vi "xnet_canopen_create.vi"(8 "error in (no error)":errorcluster) -> (0 "error out":errorcluster, 3 "xnet_co_handle":u64)   [LabVIEW 2023, in "xnet_canopen.lvlib"]
uses:
  xnet_canopen.lvlib
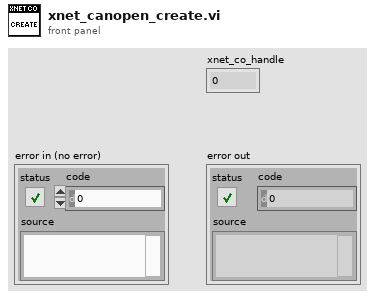
[diagram p1: front panel]
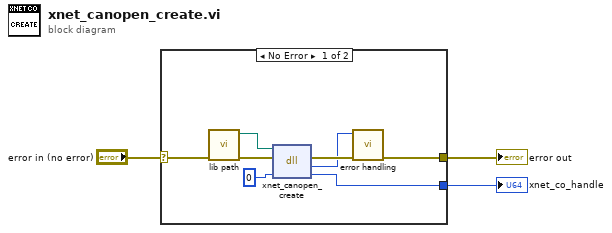
[diagram p0: block diagram]
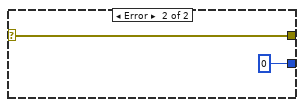
[diagram p2: hidden frame]
diagram:
  n1 = case shown="No Error" "error in (no error)" {
    selector: "error in (no error)" -> [w8 w12]
    tunnel: [w6 w12] -> w2
    tunnel: [w4 u64 0 ("phandle")] -> w1
    frame No Error {
      n2 = call "lib path.vi"() -> ("lib path"=w10:path)  [unwired: 11 in]
      n3 = dll-call lib="?" fn="xnet_canopen_create"(path in=w10, error in=w8, "phandle"=u64 0) -> (error out=w7:errorcluster, "return type"=w5:i32, "phandle"=w4:u64)  [unwired: 1 in, 1 out]
      n4 = call "error handling.vi"("error in (no error)"=w7, "return val"=w5) -> ("error out"=w6:errorcluster)  [unwired: 9 in]
    }
    frame Error {
    }
  }
  "error out" <- w2
  "xnet_co_handle" <- w1
